vi "Read number total including repeat.vi"(8 "noise MAX":i32=3, 11 "Read No":i32[](array[numeric])) -> (0 "AR %":dbl[](array[numeric]), 1 "AR N#":i32[](array[numeric]), 2 "AR T#":i32, 3 "シグナル集計":dbl[][](array[numeric]), 4 "平均 Read N":dbl format="%#_4g", 5 "MAX_R#":i32, 6 "Av n#":dbl, 7 "AR BN#":i32[](array[numeric]), 10 "Av n#bp":i32)   [LabVIEW 2018]
panel:
  out "数値 3":i32
  out "数値 2":i32
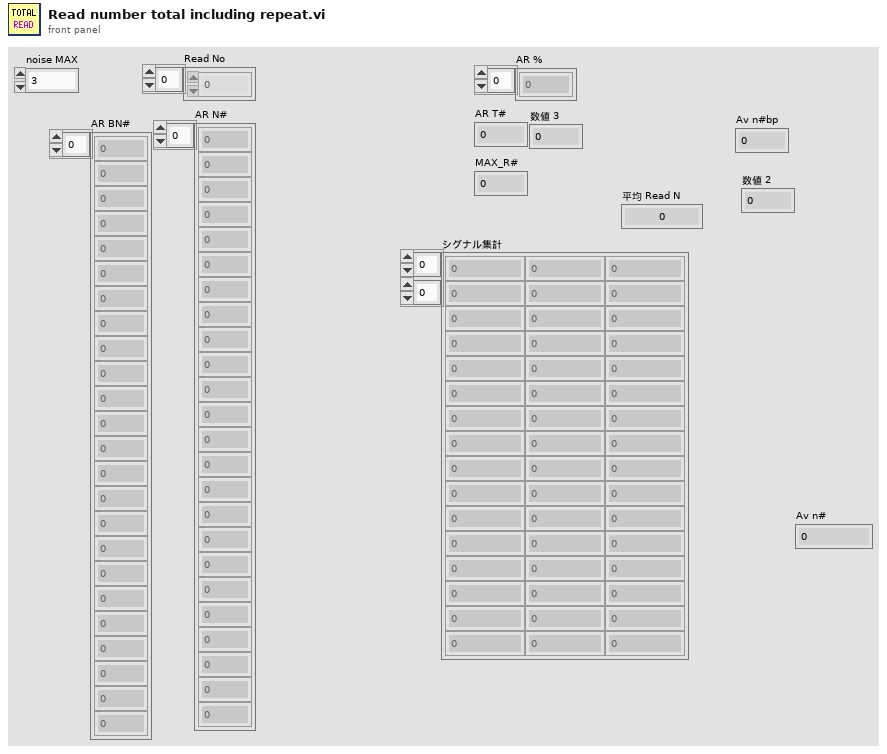
[diagram p1: front panel]
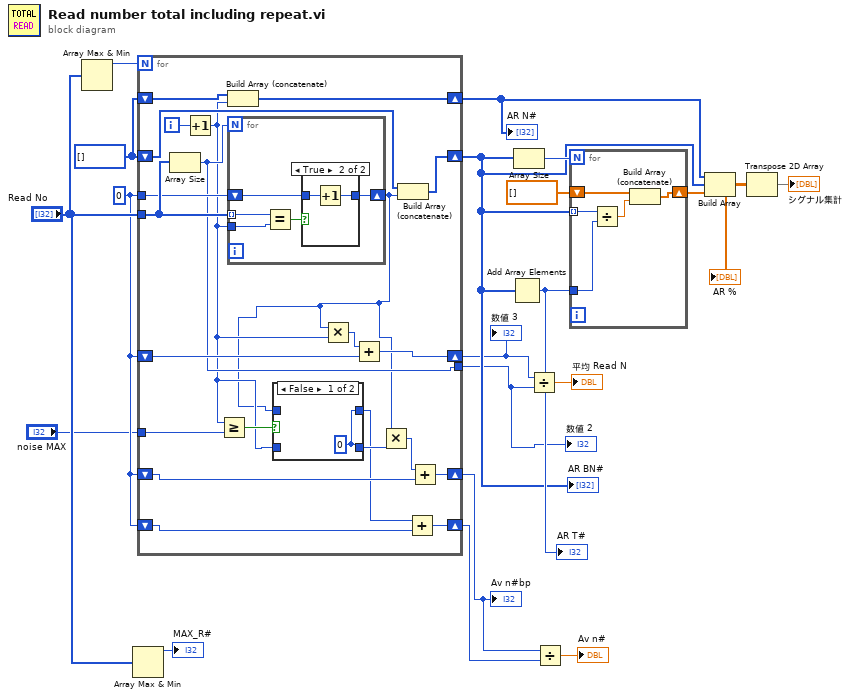
[diagram p0: block diagram]
diagram:
  w3 = 0
  w19 = i32[] []
  n1 = Array Max & Min(array="Read No") -> (max value=w20:i32)  [unwired: 3 out]
  n2 = Array Max & Min(array="Read No") -> (max value=→"MAX_R#":i32)  [unwired: 3 out]
  n3 = for {
    N: w20 -> [_]
    tunnel: "Read No" -> [w42]
    tunnel: w3 -> [w40]
    shift-right: [w39] -> w12
    shift-left: w19 -> [w38]
    shift-right: [w37] -> w11
    shift-left: w19 -> [w36]
    shift-right: [w33] -> w9
    shift-left: w3 -> [w34]
    tunnel: [w32] -> w5
    shift-right: [w30] -> w6
    shift-left: w3 -> [w29]
    shift-right: [w26] -> w2
    shift-left: w3 -> [w25]
    tunnel: "noise MAX" -> [w21]
    i -> [w41]
    n4 = Array Size(array=w42) -> (size(s)=w32:i32)
    n5 = Increment(x=w41) -> (x+1=w27:i32)
    n6 = Greater Or Equal?(x=w27, y=w21) -> (x >= y?=w28:bool)
    n7 = Build Array (concatenate)(w36, w27) -> (w37:i32[])
    n8 = for {
      N: w32 -> [_]
      tunnel: w42 -> [w48] mode=indexing
      tunnel: w27 -> [w49]
      shift-right: [w46] -> w23
      shift-left: w40 -> [w47]
      n9 = Equal?(x=w48, y=w49) -> (x = y?=w50:bool)
      n10 = case shown="True" w50 {
        tunnel: [w51 w53] -> w46
        tunnel: w47 -> [w51 w52]
        frame False {
        }
        frame True {
          n11 = Increment(x=w52) -> (x+1=w53:i32)
        }
      }
    }
    n12 = case shown="False" w28 {
      tunnel: w27 -> [_ w45]
      tunnel: [w43 w45] -> w24
      tunnel: w23 -> [_ w44]
      tunnel: [w43 w44] -> w22
      frame False {
        w43 = 0
      }
      frame True {
      }
    }
    n13 = Multiply(x=w23, y=w27) -> (x*y=w35:i32)
    n14 = Add(x=w35, y=w34) -> (x+y=w33:i32)
    n15 = Multiply(x=w23, y=w24) -> (x*y=w31:i32)
    n16 = Build Array (concatenate)(w38, w23) -> (w39:i32[])
    n17 = Add(x=w22, y=w25) -> (x+y=w26:i32)
    n18 = Add(x=w31, y=w29) -> (x+y=w30:i32)
  }
  "AR BN#" <- w12
  "AR N#" <- w11
  "Av n#bp" <- w6
  "数値 2" <- w5
  "数値 3" <- w9
  n19 = Add Array Elements(numeric array=w12) -> (sum=w18:i32)
  "AR T#" <- w18
  n20 = Array Size(array=w12) -> (size(s)=w17:i32)
  n21 = Divide(x=w9, y=w5) -> (x/y=→"平均 Read N":dbl)
  n22 = Divide(x=w6, y=w2) -> (x/y=→"Av n#":dbl)
  n23 = for {
    N: w17 -> [_]
    tunnel: w12 -> [w58] mode=indexing
    tunnel: w18 -> [w57]
    shift-right: [w55] -> w13
    shift-left: dbl[] [] -> [w54]
    n24 = Divide(x=w58, y=w57) -> (x/y=w56:dbl)
    n25 = Build Array (concatenate)(w54, w56) -> (w55:dbl[])
  }
  "AR %" <- w13
  n26 = Build Array(w11, w12, w13) -> (w15:dbl[][])
  n27 = Transpose 2D Array(2D array=w15) -> (transposed array=→"シグナル集計":dbl[][])
